vi "set RBW or VBW.vi"(6 "BW Auto?":bool, 8 "error in (no error)":errorcluster, 9 "BW Type":T1, 10 "BW Value (Hz)":dbl format="%#_6p", 11 "FSV-40N in":refnum<class "FSV-40N.lvclass">) -> (0 "error out":errorcluster, 3 "FSV-40N out":refnum<class "FSV-40N.lvclass">)   [LabVIEW 2023, in "Spectrum Analyzer.lvlib" / "FSV-40N.lvclass"]
uses:
  FSV-40N.lvclass
  TYPE DEFINITION/TYPE RBW and VBW Select.ctl
  FSV-40N.lvclass/FSV-40N.ctl
  Spectrum Analyzer.lvlib
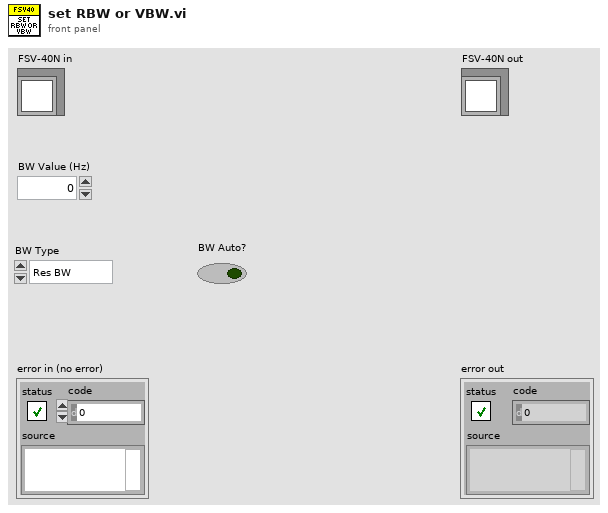
[diagram p1: front panel]
types:
  T1 = typedef "Spectrum Analyzer.lvlib/TYPE RBW and VBW Select.ctl" = enum16{"Res BW", "Video BW"}
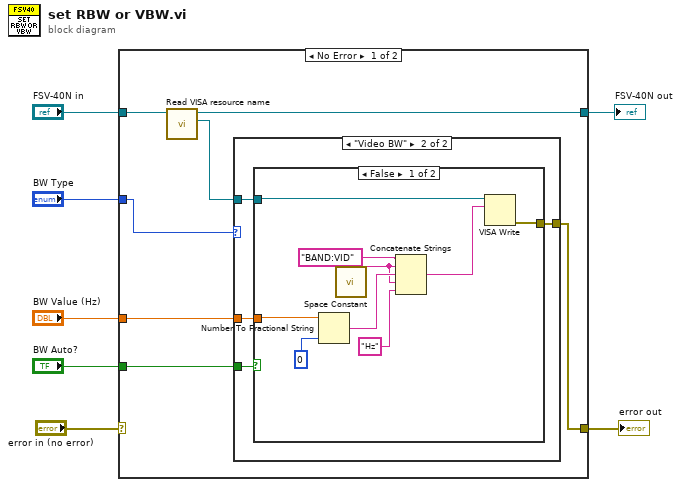
[diagram p0: block diagram]
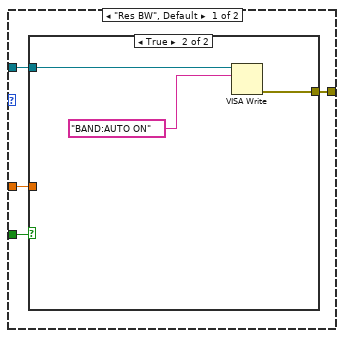
[diagram p2: hidden frame]
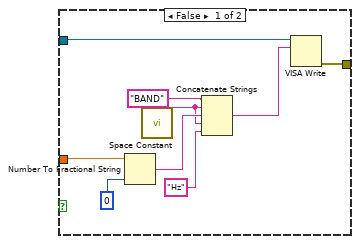
[diagram p3: hidden frame]
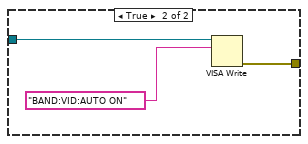
[diagram p4: hidden frame]
diagram:
  n1 = case shown="No Error" "error in (no error)" {
    selector: "error in (no error)" -> [_ w47]
    tunnel: "FSV-40N in" -> [w14 w48]
    tunnel: [w13 w48] -> w5
    tunnel: [w8 w47] -> w4
    tunnel: "BW Type" -> [w11 _]
    tunnel: "BW Auto?" -> [w10 _]
    tunnel: "BW Value (Hz)" -> [w9 _]
    frame No Error {
      n2 = call "Read VISA resource name.vi"("FSV-40N in"=w14) -> ("VISA resource name"=w12:refnum<visa-resource-name>, "FSV-40N out"=w13:refnum<class "FSV-40N.lvclass">)  [unwired: 8 in, 1 out]
      n3 = case shown="\"Video BW\"" w11 {
        tunnel: w12 -> [w17 w33]
        tunnel: w10 -> [w18 w34]
        tunnel: [w16 w32] -> w8
        tunnel: w9 -> [w15 w31]
        frame "Res BW", Default {
          n4 = case shown="True" w18 {
            tunnel: w17 -> [w27 w30]
            tunnel: [w19 w28] -> w16
            tunnel: w15 -> [w26 _]
            frame False {
              n5 = Number To Fractional String(number=w26, precision (6)=i16 0) -> (F-format string=w23:string)  [unwired: 2 in]
              n6 = call <vilib>:"Space Constant.vi"() -> ("String"=w22:string)
              n7 = Concatenate Strings("BAND" ("string"), w22, w23, w22, "Hz" ("string")) -> (w20:string)
              n8 = VISA Write(VISA resource name=w27, write buffer=w20) -> (error out=w19:errorcluster)  [unwired: 1 in, 2 out]
            }
            frame True {
              n9 = VISA Write(VISA resource name=w30, write buffer="BAND:AUTO ON") -> (error out=w28:errorcluster)  [unwired: 1 in, 2 out]
            }
          }
        }
        frame "Video BW" {
          n10 = case shown="False" w34 {
            tunnel: w33 -> [w43 w46]
            tunnel: [w35 w44] -> w32
            tunnel: w31 -> [w42 _]
            frame False {
              n11 = Number To Fractional String(number=w42, precision (6)=i16 0) -> (F-format string=w39:string)  [unwired: 2 in]
              n12 = call <vilib>:"Space Constant.vi"() -> ("String"=w38:string)
              n13 = Concatenate Strings("BAND:VID" ("string"), w38, w39, w38, "Hz" ("string")) -> (w36:string)
              n14 = VISA Write(VISA resource name=w43, write buffer=w36) -> (error out=w35:errorcluster)  [unwired: 1 in, 2 out]
            }
            frame True {
              n15 = VISA Write(VISA resource name=w46, write buffer="BAND:VID:AUTO ON") -> (error out=w44:errorcluster)  [unwired: 1 in, 2 out]
            }
          }
        }
      }
    }
    frame Error {
    }
  }
  "error out" <- w4
  "FSV-40N out" <- w5
